vi "LADAR value save VI.vi"(8 "error in":errorcluster caption="エラー入力（エラーなし）", 9 "LL_Base_Com_Array":i32[](array[numeric]), 10 "LL_Base Tag_Array":string[](array[string]), 11 "TDMSファイル入力":refnum<k34>) -> (0 "error out":errorcluster caption="エラー出力", 3 "A TDMSファイル出力":refnum<k34>)   [LabVIEW 2018]
panel:
  out "decimal integer string":string[](array[string])
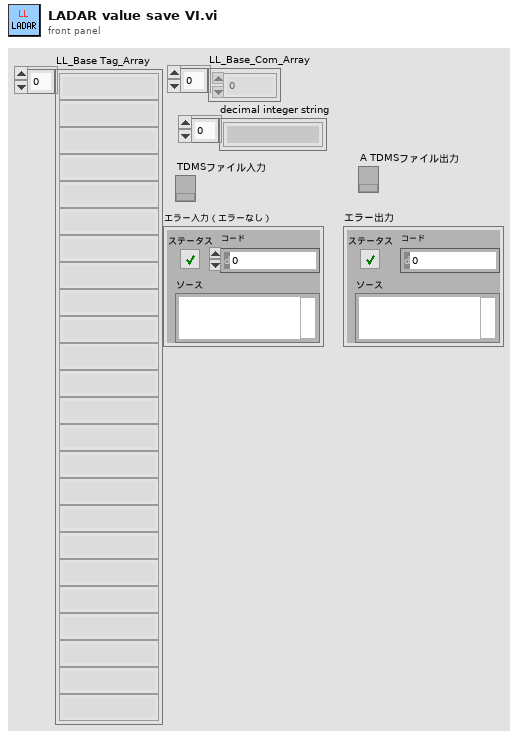
[diagram p1: front panel]
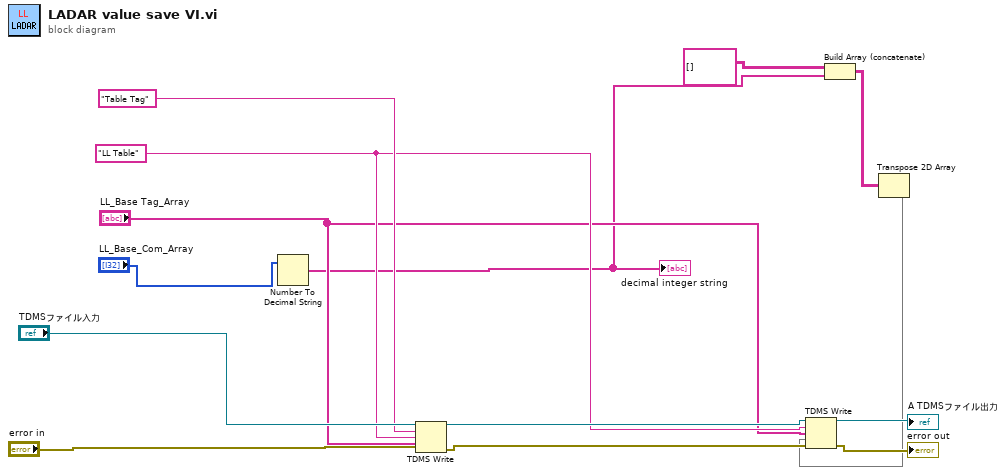
[diagram p0: block diagram]
diagram:
  w7 = "LL Table" ("チャンネル名入力（名称未設定）")
  n1 = Number To Decimal String(number="LL_Base_Com_Array") -> (decimal integer string=w3:string[])  [unwired: 1 in]
  "decimal integer string" <- w3
  n2 = TDMS Write(0:"TDMSファイル入力", 5:"Table Tag" ("グループ名入力（名称未設定）"), 7:w7, 9:"LL_Base Tag_Array", 11:"error in") -> (4:w8:refnum<k34>, 15:w9:errorcluster)  [unwired: 1 in, 2 out]
  n3 = Build Array (concatenate)(string[][] [] ("Table"), w3) -> (w2:string[][])
  n4 = Transpose 2D Array(2D array=w2) -> (transposed array=w1:string[][])
  n5 = TDMS Write(0:w8, 5:w7, 7:"LL_Base Tag_Array", 9:w1, 11:w9) -> (4:→"A TDMSファイル出力":refnum<k34>, 15:→"error out":errorcluster)  [unwired: 1 in, 2 out]
